vi "Iterate.vi"(8 "error in (no error)":errorcluster, 11 "Example Actor in":refnum<class "Example Actor.lvclass">) -> (0 "error out":errorcluster, 3 "Example Actor out":refnum<class "Example Actor.lvclass">)   [LabVIEW 2023, in "Example Iterator NR Actor.lvlib" / "Example Actor.lvclass"]
doc: "Method called duriong the iterations"
uses:
  Example Actor.lvclass
  Example Actor.lvclass/Example Actor.ctl
  <userlib>/_OpenG.lib/time/time.llb/openg_time.lvlib
  Iterator NR Actor Messages/Break Msg/Break Msg.lvclass
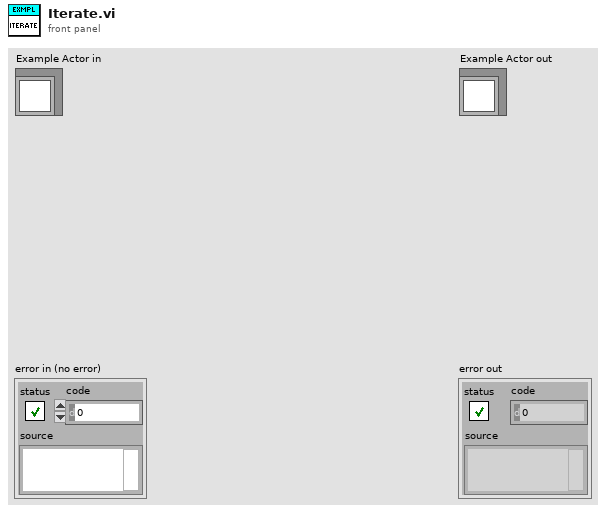
[diagram p1: front panel]
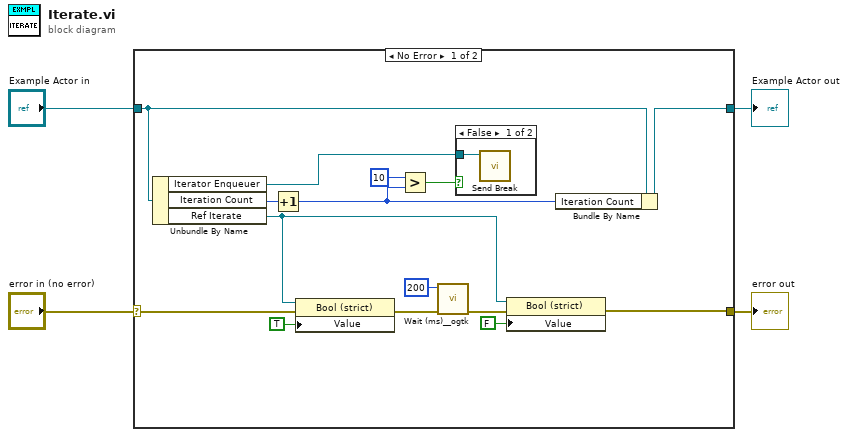
[diagram p0: block diagram]
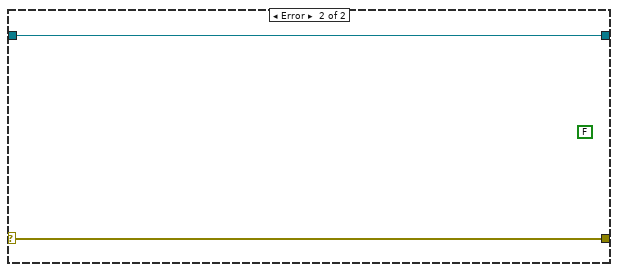
[diagram p3: hidden frame]
diagram:
  n1 = case shown="No Error" "error in (no error)" {
    selector: "error in (no error)" -> [w18 w22]
    tunnel: [w11 w22] -> w3
    tunnel: [w9 w21] -> w1
    tunnel: "Example Actor in" -> [w19 w21]
    frame No Error {
      n2 = Unbundle By Name(w19) -> ("Iterator Enqueuer"=w6:refnum<class "Message Enqueuer.lvclass">, "Iteration Count"=w10:i32, "Ref Iterate"=w15:refnum<vi>)
      n3 = Increment(x=w10) -> (x+1=w8:i32)
      n4 = property class="Bool (strict)"(reference=w15, error in=w18, "Value"=TRUE) -> (error out=w17:errorcluster)  [unwired: 1 out]
      n5 = Greater?(x=10, y=w8) -> (0:w5:bool)
      n6 = call <userlib>:"Wait (ms)__ogtk.vi"("error in (no error)"=w17, "milliseconds to wait"=u32 200) -> ("error out"=w16:errorcluster)  [unwired: 8 in, 1 out]
      n7 = case shown="False" w5 {
        tunnel: w6 -> [w20 _]
        frame False {
          n8 = call "Send Break.vi"("Message Enqueuer in"=w20) -> ()  [unwired: 9 in, 2 out]
        }
        frame True {
        }
      }
      n9 = property class="Bool (strict)"(reference=w15, error in=w16, "Value"=FALSE) -> (error out=w11:errorcluster)  [unwired: 1 out]
      n10 = Bundle By Name(cluster=w19, "Iteration Count"=w8) -> (w9:refnum<class "Example Actor.lvclass">)
    }
    frame Error {
      (unwired) FALSE
    }
  }
  "error out" <- w3
  "Example Actor out" <- w1
